vi "[ce] CalcExpress Routine - Error Handler.vi"(6 "error in":errorcluster, 7 "error msg":string, 9 "error code":i32=42) -> (0 "error out":errorcluster)   [LabVIEW 2021]
doc: "::: CalcExpress Toolkit :::\nCopyright (c) 2000-2026 Konstantin Shifershteyn. All rights reserved."
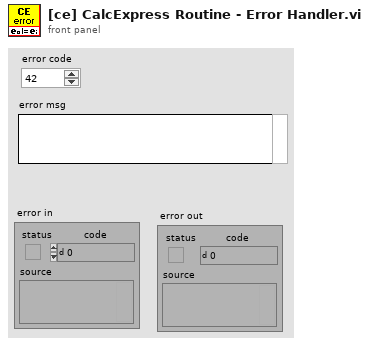
[diagram p1: front panel]
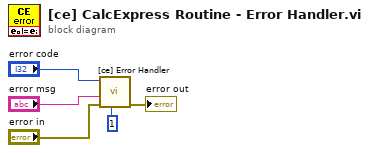
[diagram p0: block diagram]
diagram:
  n1 = call "[ce] Error Handler.vi"("nesting level"=1, "error in"="error in", "error reason"="error msg", "error code"="error code") -> ("error out"=→"error out":errorcluster)  [unwired: 6 in, 1 out]
